vi "Cron Weekdays.vi"(7 "Cron":refnum<class "Cron.lvclass">, 10 "Cron":T1) -> (2 "Cron Time":T1)   [LabVIEW 2013, in "openCron.lvlib" / "Cron.lvclass"]
uses:
  Cron.lvclass
  CronTime -- cluster.ctl
  Cron Interval -- enum.ctl
  Cron.lvclass/Cron.ctl
  <vilib>/LabVIEW Open Source Project/Epoch Date & Time/GregorianCal_Month -- enum.ctl
  <vilib>/LabVIEW Open Source Project/Epoch Date & Time/GregorianCal_MonthLengths.vi
  TimeStamp to Cron Time.vi
  Cron Time to TimeStamp.vi
  <vilib>/LabVIEW Open Source Project/Epoch Date & Time/isLeapYear (integer).vi
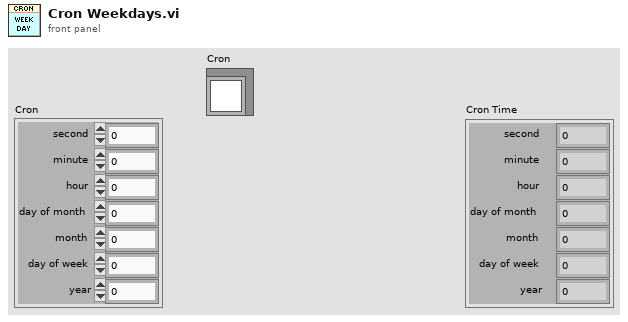
[diagram p1: front panel]
types:
  T1 = typedef "openCron.lvlib/Cron.lvclass/CronTime -- cluster.ctl" = cluster{"second":i32, "minute":i32, "hour":i32, "day of month":i32, "month":i32, "day of week":i32, "year":i32}
  T2 = typedef "openCron.lvlib/Cron.lvclass/Cron Interval -- enum.ctl" = enum16{"Seconds", "Minutes", "Hours", "Day of Month", "Month", "Day of Week", "Year"}
  T3 = typedef "openCron.lvlib/Cron.lvclass/Cron Interval -- cluster.ctl" = cluster{"Values":i32[], "All":bool, "Any":bool}
  T4 = typedef "GregorianCal_Month -- enum.ctl" = enum16{"January", "February", "March", "April", "May", "June", "July", "August", "September", "October", "November", "December"}
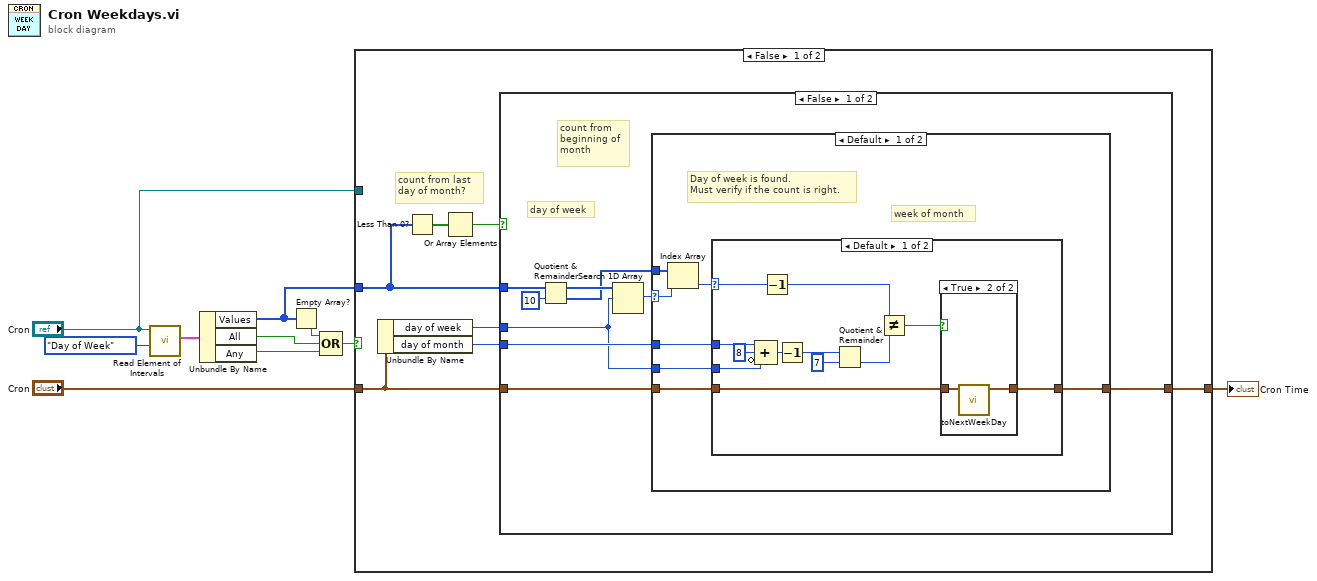
[diagram p0: block diagram]
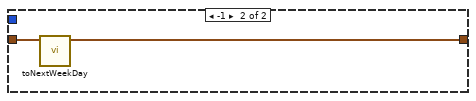
[diagram p4: hidden frame]
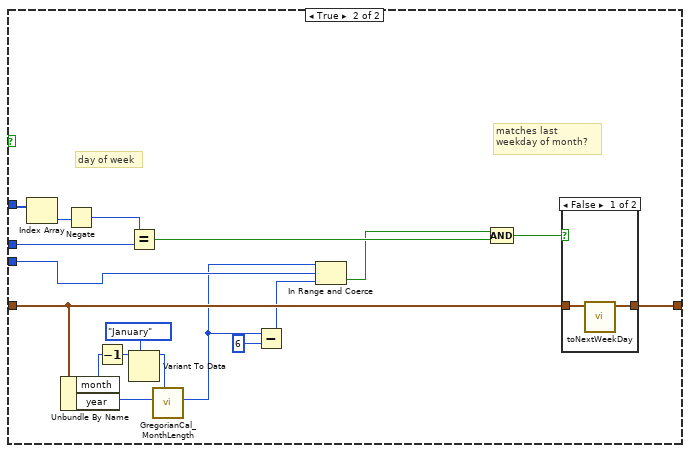
[diagram p5: hidden frame]
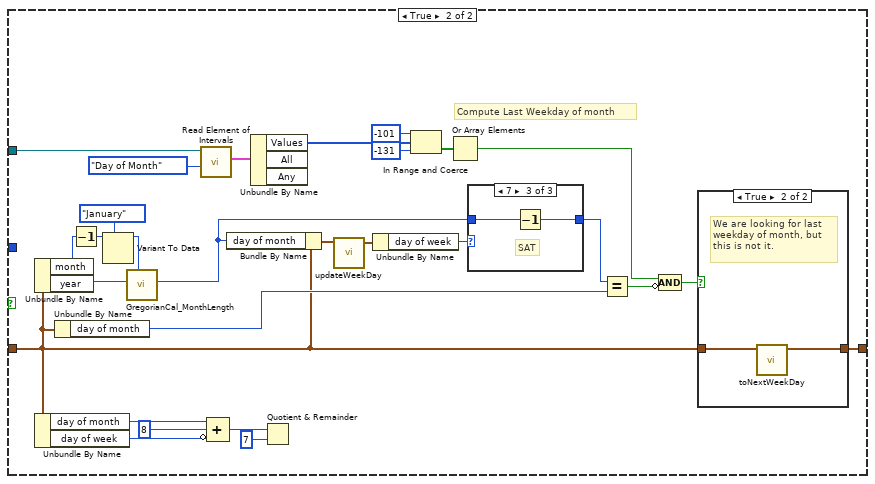
[diagram p7: hidden frame]
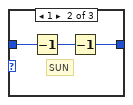
[diagram p9: hidden frame]
diagram:
  n1 = call "Read Element of Intervals.vi"("Interval"=Cron_Interval_--_enum."Day of Week", "Cron in"="Cron") -> ("Interval"=w8:T3)  [unwired: 7 in, 2 out]
  n2 = Unbundle By Name(w8) -> ("Values"=w3:i32[], "All"=w6:bool, "Any"=w7:bool)
  n3 = Empty Array?(array=w3) -> (empty?=w5:bool)
  n4 = Compound Arithmetic op=OR(w5, w6, w7) -> (w4:bool)
  n5 = case shown="False" w4 {
    tunnel: [w16 w95] -> w10
    tunnel: "Cron" -> [w17 w85]
    tunnel: w3 -> [w13 _]
    tunnel: "Cron" -> [_ w75]
    frame False {
      # "count from last \nday of month?"
      n6 = Unbundle By Name(w17) -> ("day of week"=w14:i32, "day of month"=w15:i32)
      n7 = Less Than 0?(x=w13) -> (x < 0?=w12:bool[])
      n8 = Or Array Elements(Boolean array=w12) -> (logical OR=w11:bool)
      n9 = case shown="False" w11 {
        tunnel: w17 -> [w26 w69]
        tunnel: [w25 w68] -> w16
        tunnel: w15 -> [w20 w55]
        tunnel: w14 -> [w19 w60]
        tunnel: w13 -> [w18 w67]
        frame False {
          # "day of week"
          # "count from\nbeginning of\nmonth"
          n10 = Quotient & Remainder(x=w18, y=10) -> (x-y*floor(x/y)=w22:i32[], floor(x/y)=w21:i32[])
          n11 = Search 1D Array(1D array=w22, element=w19) -> (index of element=w24:i32)  [unwired: 1 in]
          n12 = case shown="Default" w24 {
            selector: w24 -> [w33 _]
            tunnel: w26 -> [w28 w51]
            tunnel: [w32 w50] -> w25
            tunnel: w21 -> [w29 _]
            tunnel: w20 -> [w31 _]
            tunnel: w19 -> [w30 _]
            frame Default {
              # "Day of week is found.\nMust verify if the count is right."
              # "week of month"
              n13 = Index Array(array=w29, index=w33) -> (element=w27:i32)
              n14 = case shown="Default" w27 {
                selector: w27 -> [w36 _]
                tunnel: [w45 w49] -> w32
                tunnel: w31 -> [w41 _]
                tunnel: w30 -> [w40 _]
                tunnel: w28 -> [w39 w49]
                frame Default {
                  n15 = Compound Arithmetic op=ADD(w41, 8 ("value"), invert w40) -> (w42:i32)
                  n16 = Decrement(x=w36) -> (x-1=w35:i32)
                  n17 = Decrement(x=w42) -> (x-1=w34:i32)
                  n18 = Quotient & Remainder(x=w34, y=7) -> (floor(x/y)=w38:i32)  [unwired: 1 out]
                  n19 = Not Equal?(x=w35, y=w38) -> (x != y?=w37:bool)
                  n20 = case shown="True" w37 {
                    tunnel: w39 -> [w46 w48]
                    tunnel: [w46 w47] -> w45
                    frame False {
                    }
                    frame True {
                      n21 = call "toNextWeekDay.vi"("Cron in"=w48) -> ("Cron out"=w47:T1)  [unwired: 10 in]
                    }
                  }
                }
                frame 0 {
                }
              }
            }
            frame -1 {
              n22 = call "toNextWeekDay.vi"("Cron in"=w51) -> ("Cron out"=w50:T1)  [unwired: 10 in]
            }
          }
        }
        frame True {
          # "matches last\nweekday of month?"
          # "day of week"
          n23 = Index Array(array=w67) -> (element=w66:i32)  [unwired: 1 in]
          n24 = Unbundle By Name(w69) -> ("month"=w62:i32, "year"=w61:i32)
          n25 = Negate(x=w66) -> (-x=w59:i32)
          n26 = Decrement(x=w62) -> (x-1=w65:i32)
          n27 = Equal?(x=w59, y=w60) -> (x = y?=w58:bool)
          n28 = Variant To Data(type=GregorianCal_Month_--_enum."January" ("Month"), Variant=w65) -> (data=w64:T4)  [unwired: 1 in, 1 out]
          n29 = call <vilib>:"GregorianCal_MonthLength.vi"("Month"=w64, "Year (0: this year)"=w61) -> ("Nb Days"=w53:i32)  [unwired: 9 in]
          n30 = Subtract(x=w53, y=6) -> (x-y=w54:i32)
          n31 = In Range and Coerce(upper limit=w53, x=w55, lower limit=w54) -> (In Range?=w52:bool)  [unwired: 1 out]
          n32 = Compound Arithmetic op=AND(w52, w58) -> (w57:bool)
          n33 = case shown="False" w57 {
            tunnel: w69 -> [w71 w72]
            tunnel: [w70 w72] -> w68
            frame False {
              n34 = call "toNextWeekDay.vi"("Cron in"=w71) -> ("Cron out"=w70:T1)  [unwired: 10 in]
            }
            frame True {
            }
          }
        }
      }
    }
    frame True {
      # "Compute Last Weekday of month"
      n35 = Unbundle By Name(w85) -> ("month"=w97:i32, "year"=w96:i32)
      n36 = Unbundle By Name(w85) -> ("day of month"=w91:i32, "day of week"=w90:i32)
      n37 = Unbundle By Name(w85) -> ("day of month"=w89:i32)
      n38 = Decrement(x=w97) -> (x-1=w100:i32)
      n39 = Variant To Data(type=GregorianCal_Month_--_enum."January" ("Month"), Variant=w100) -> (data=w99:T4)  [unwired: 1 in, 1 out]
      n40 = call <vilib>:"GregorianCal_MonthLength.vi"("Month"=w99, "Year (0: this year)"=w96) -> ("Nb Days"=w81:i32)  [unwired: 9 in]
      n41 = call "Read Element of Intervals.vi"("Interval"=Cron_Interval_--_enum."Day of Month", "Cron in"=w75) -> ("Interval"=w76:T3)  [unwired: 7 in, 2 out]
      n42 = Compound Arithmetic op=ADD(w91, 8 ("value"), invert w90) -> (w92:i32)
      n43 = Bundle By Name(cluster=w85, "day of month"=w81) -> (w84:T1)
      n44 = Unbundle By Name(w76) -> ("Values"=w73:i32[])  [unwired: 2 out]
      n45 = Quotient & Remainder(x=w92, y=7) -> ()  [unwired: 2 out]
      n46 = call "updateWeekDay.vi"("Cron in"=w84) -> ("Cron Time"=w83:T1)  [unwired: 10 in]
      n47 = Unbundle By Name(w83) -> ("day of week"=w82:i32)
      n48 = In Range and Coerce(upper limit=-101, x=w73, lower limit=-131) -> (In Range?=w77:bool[])  [unwired: 1 out]
      n49 = Or Array Elements(Boolean array=w77) -> (logical OR=w88:bool)
      n50 = case shown="7" w82 {
        tunnel: [w101 w102 w105] -> w80
        tunnel: w81 -> [w101 w104 w106]
        frame Default {
          # "MON-FRI"
        }
        frame 1 {
          # "SUN"
          n51 = Decrement(x=w104) -> (x-1=w103:i32)
          n52 = Decrement(x=w103) -> (x-1=w102:i32)
        }
        frame 7 {
          # "SAT"
          n53 = Decrement(x=w106) -> (x-1=w105:i32)
        }
      }
      n54 = Equal?(x=w80, y=w89) -> (x = y?=w87:bool)
      n55 = Compound Arithmetic op=AND(w88, invert w87) -> (w86:bool)
      n56 = case shown="True" w86 {
        tunnel: w85 -> [w107 w109]
        tunnel: [w107 w108] -> w95
        frame False {
        }
        frame True {
          # "We are looking for last\nweekday of month, but\nthis is not it."
          n57 = call "toNextWeekDay.vi"("Cron in"=w109) -> ("Cron out"=w108:T1)  [unwired: 10 in]
        }
      }
    }
  }
  "Cron Time" <- w10
